vi "Set GPIO Pull.vi"(8 "error in (no error)":errorcluster, 10 "GPIO Pull":T1, 11 "CTI_GPIO_DigitalOut in":refnum<class "CTI_GPIO_DigitalOut.lvclass">) -> (0 "error out":errorcluster, 3 "CTI_GPIO_DigitalOut out":refnum<class "CTI_GPIO_DigitalOut.lvclass">)   [LabVIEW 2021, in "CTI_GPIO_DigitalOut.lvclass"]
uses:
  CTI_GPIO_DigitalOut.lvclass
  <vilib>/CTI/CTI Drivers/CTI/GPIO Pull.ctl
  CTI_GPIO_DigitalOut.lvclass/CTI_GPIO_DigitalOut.ctl
  <vilib>/CTI/CTI Drivers/CTI/CTI.lvlib
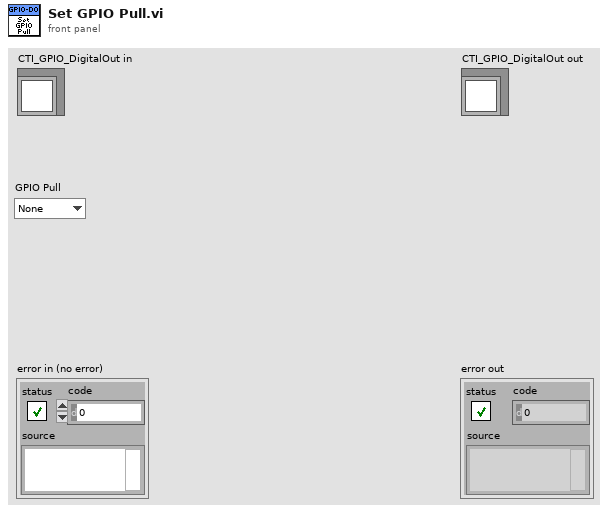
[diagram p1: front panel]
types:
  T1 = typedef "CTI.lvlib/GPIO Pull.ctl" = enum16{"None", "Up", "Down", "Both"}
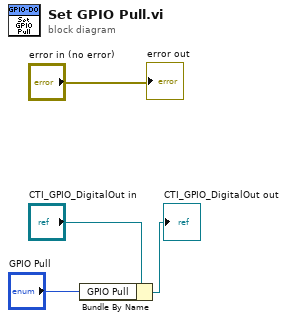
[diagram p0: block diagram]
diagram:
  n1 = Bundle By Name(cluster="CTI_GPIO_DigitalOut in", "GPIO Pull"="GPIO Pull") -> (→"CTI_GPIO_DigitalOut out":refnum<class "CTI_GPIO_DigitalOut.lvclass">)
  "error out" <- "error in (no error)"
